vi "mupExpr Multi Test.vi"() -> ()   [LabVIEW 2015]
uses:
  mupExpr/mupExpr.lvclass/mupExpr.ctl
  mupExpr/SetVarVal.vi
  mupLib/mupEval.vi
  mupLib/mupSetVarValue.vi
  mupLib/mupCheckError.vi
  mupLib/mupLibPath.vi
  <vilib>/Utility/error.llb/Error Cluster From Error Code.vi
  mupExpr/mupExpr.lvclass
panel:
  out "Array":dbl[][](array[numeric])
  out "Instance":i32
  out "Result":dbl
  out "error out":errorcluster
  in  "Instances":i32=10
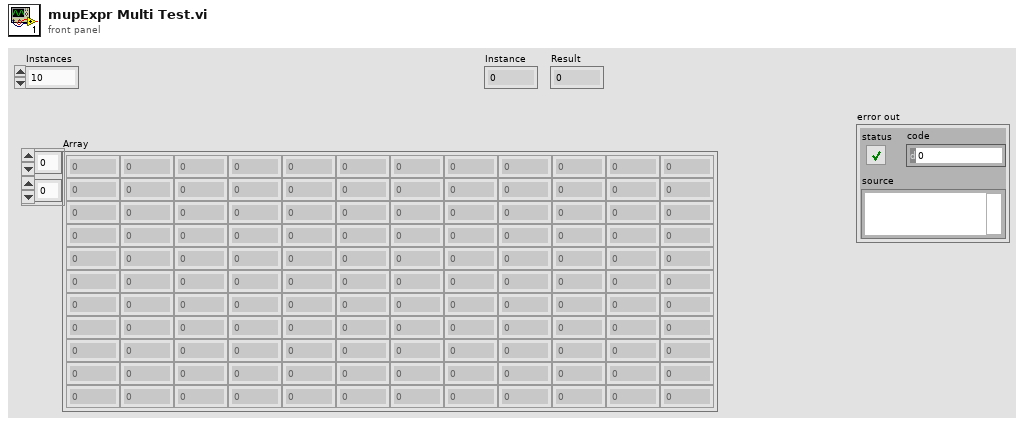
[diagram p1: front panel]
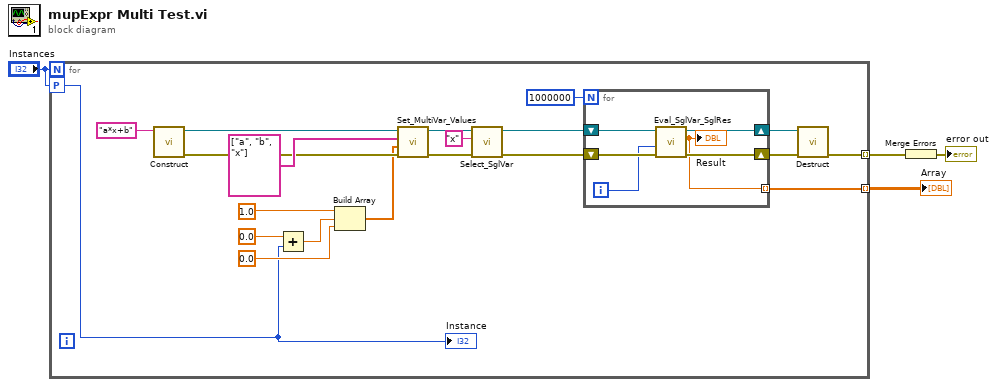
[diagram p0: block diagram]
diagram:
  n1 = for {
    N: "Instances" -> [_]
    tunnel: [w7] -> w3 mode=indexing
    workers-P: "Instances" -> [w5]
    tunnel: [w6] -> w2 mode=indexing
    n2 = call "Construct.vi"("Expression"="a*x+b") -> ("error out"=w21:errorcluster, "mupExpr out"=w23:refnum<data-value>)  [unwired: 8 in, 1 out]
    n3 = Add(x=0.0, y=w5) -> (x+y=w18:dbl)
    n4 = Build Array(1.0, w18, 0.0) -> (w16:dbl[])
    n5 = call "Set_MultiVar_Values.vi"("error in (no error)"=w21, "varValues"=w16, "varNames"=string[] ["a", "b", "x"], "mupExpr in"=w23) -> ("error out"=w14:errorcluster, "mupExpr out"=w15:refnum<data-value>)  [unwired: 6 in]
    n6 = call "Select_SglVar.vi"("error in (no error)"=w14, "varName"="x", "mupExpr in"=w15) -> ("error out"=w10:errorcluster, "mupExpr out"=w11:refnum<data-value>)  [unwired: 7 in]
    n7 = for {
      N: 1000000 -> [_]
      shift-right: [w27] -> w9
      shift-left: w11 -> [w30]
      shift-right: [w28] -> w8
      shift-left: w10 -> [w29]
      tunnel: [w25] -> w6 mode=indexing
      i -> [w26]
      n8 = call "Eval_SglVar_SglRes.vi"("error in (no error)"=w29, "varValue"=w26, "mupExpr in"=w30) -> ("error out"=w28:errorcluster, "Result"=w25:dbl, "mupExpr out"=w27:refnum<data-value>)  [unwired: 6 in]
      "Result" <- w25
    }
    n9 = call "Destruct.vi"("error in (no error)"=w8, "mupExpr in"=w9) -> ("error out"=w7:errorcluster)  [unwired: 9 in]
    "Instance" <- w5
  }
  "Array" <- w2
  n10 = Merge Errors(w3) -> (→"error out":errorcluster)
